vi "Get Collect Times.vi"(8 "error in (no error)":errorcluster caption="错误输入（无错误）", 10 "uColloctionTimes":cluster{} caption="空簇", 11 "nDevId":i32) -> (0 "error out":errorcluster caption="错误输出", 2 "uColloctionTimes out":cluster{} caption="空簇", 3 "function return":i32)   [LabVIEW 2017, in "smncsftmt.lvlib"]
doc: "__declspec(dllexport) int GetCollectTimes(int nDevId, unsigned long long* uColloctionTimes);"
uses:
  smncsftmt.lvlib
  smncsftmt.dll
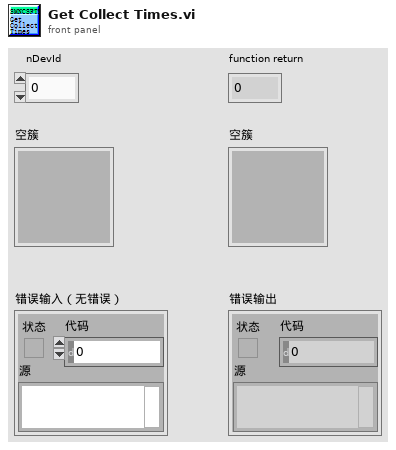
[diagram p1: front panel]
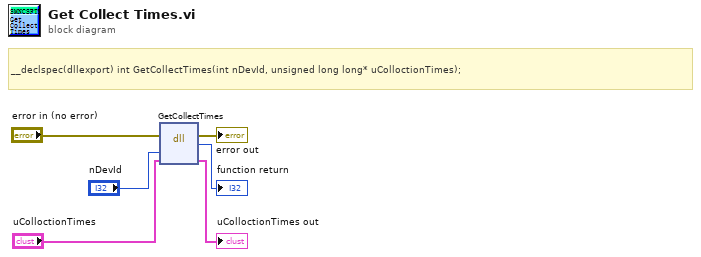
[diagram p0: block diagram]
diagram:
  # "__declspec(dllexport) int GetCollectTimes(int nDevId, unsigned long long* uColloctionTimes);"
  n1 = dll-call lib="PTH2oabs CUsersaDesktop\nLABVIEW范例National InstrumentsLabVIEW 2017user.lib\tsmncsftmtsmncsftmt.*" fn="GetCollectTimes"(error in="error in (no error)", "nDevId"="nDevId", "uColloctionTimes"="uColloctionTimes") -> (error out=→"error out":errorcluster, →"function return":i32, "uColloctionTimes"=→"uColloctionTimes out":cluster{})  [unwired: 3 in, 1 out]
